vi "midiOutOpen.vi"(8 "error in":errorcluster, 10 "DeviceID":u32, 11 "midi in":refnum<class "midi.lvclass">) -> (0 "error out":errorcluster, 3 "midi out":refnum<class "midi.lvclass">)   [LabVIEW 2020, in "midi.lvclass"]
doc: "The midiOutOpen function opens a MIDI output device for playback."
uses:
  midi.lvclass
  midi.lvclass/midi.ctl
  winmm.dll
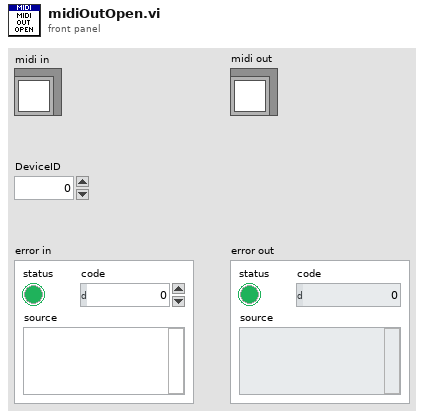
[diagram p1: front panel]
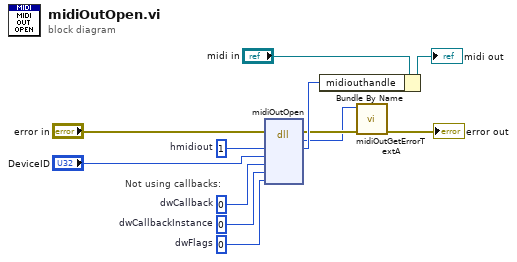
[diagram p0: block diagram]
diagram:
  w7 = 0  # dwFlags
  w8 = 0  # dwCallbackInstance
  w9 = 0  # dwCallback
  w10 = u64 1  # hmidiout
  # "Not using callbacks:"
  n1 = dll-call lib="winmm.dll" fn="midiOutOpen"(error in="error in", "hmidiout"=w10, "uDeviceID"="DeviceID", "dwCallback"=w9, "dwCallbackInstance"=w8, "dwFlags"=w7) -> (error out=w4:errorcluster, "return type"=w2:i32, "hmidiout"=w5:u64)  [unwired: 6 in, 1 out]
  n2 = Bundle By Name(cluster="midi in", "midiouthandle"=w5) -> (→"midi out":refnum<class "midi.lvclass">)
  n3 = call "midiOutGetErrorTextA.vi"("error in"=w4, "Error Code"=w2) -> ("error out"=→"error out":errorcluster)  [unwired: 9 in]
